vi "VIH HelpGen - Write HTML File - Poly VI.vi"(6 "Owning Palette":cluster{"Name":string, "HTML Path":path}, 8 "error in":errorcluster, 9 "HTML Path":path, 10 "VI Path":path, 11 "Project Tree":T1) -> (0 "error out":errorcluster, 3 "dup Project Tree":T1)   [LabVIEW 2014]
doc: "::: VI Helpeks :::\nCopyright (c) 2000-2026 Konstantin Shifershteyn. All rights reserved."
uses:
  _VIH Project Manager.llb/VIH Project Tree Typedef - Tree Refnum.ctl
panel:
  # "VI Helpeks\nCopyright (c) 2012-2026 Konstantin Shifershteyn"
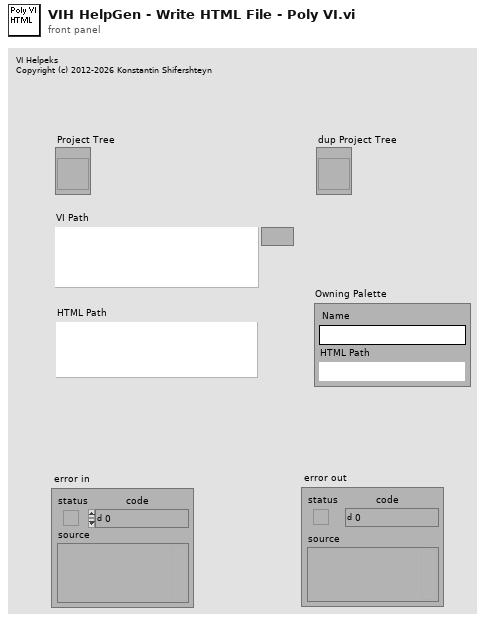
[diagram p1: front panel]
types:
  T1 = typedef "VIH Project Tree Typedef - Tree Refnum.ctl" = refnum<vi>
  T2 = typedef "VIH HelpGen Typedef - Cluster - File Rule.ctl" = cluster{"OutName":string, "BuildHelp":T3, "Source Paths":T4, "Target Paths":T5, "DscrMode":T6, "Description":string, "Control Rules":T7[], "Flags":T9, "Ctl_DscrMode":T6, "Ctl_ClustMembers":T3, "Ctl_EnumValues":T3, "MenuItemIcons":T3, "%Comments":string, "DetailsMode":T6, "DetailsText":string, "ProductInfoMode":T3, "ProductInfoText":string}
  T3 = typedef "VIH HelpGen Typedef - Enum - Default,Enable,Disable.ctl" = enum16{"Default", "Enable", "Disable"}
  T4 = typedef "VIH HelpGen Typedef - Cluster - File Rule - Source Paths.ctl" = cluster{"CSS Files":path[], "JS Files":path[], "Html Template":path}
  T5 = typedef "VIH HelpGen Typedef - Cluster - File Rule - Target Paths.ctl" = cluster{"HTML Dir":path, "Image Dir":path, "CSS Dir":path, "JS Dir":path}
  T6 = typedef "VIH HelpGen Typedef - Enum - Description Mode.ctl" = enum16{"Default", "Description", "Description1", "Description2", "Custom", "None"}
  T7 = typedef "VIH HelpGen Typedef - Cluster - Control Rule.ctl" = cluster{"CtrlID":string, "CustomRule":bool, "DscrMode":T6, "Description":string, "ClusterMembers":T3, "EnumValues":T3, "EnumValDscr":T8[], "CustomName":string}
  T8 = typedef "VIH HelpGen Typedef - Cluster - Enum Value Info.ctl" = cluster{"Value":ext, "String":string, "Description":string}
  T9 = typedef "VIH HelpGen Typedef - Cluster - Group Rule - Flags.ctl" = cluster{"Override CSS Files":bool, "Override JS Files":bool, "Override Ctl Rules":bool}
  T10 = cluster{"ProductInfoMode":T3, "ProductInfoText":string}
  T11 = typedef "VIH HelpGen Typedef - Table Templates Cluster - VI Help.ctl" = cluster{"Ctrl Dscr":string, "Ring Val Dscr":string, "Enum Val Dscr":string, "VI Details":string}
  T12 = cluster{"VI Instance Dscr":string, "Table Templates":T11}
  T13 = cluster{"directory path out":path, "directory path out":path, "name":string}
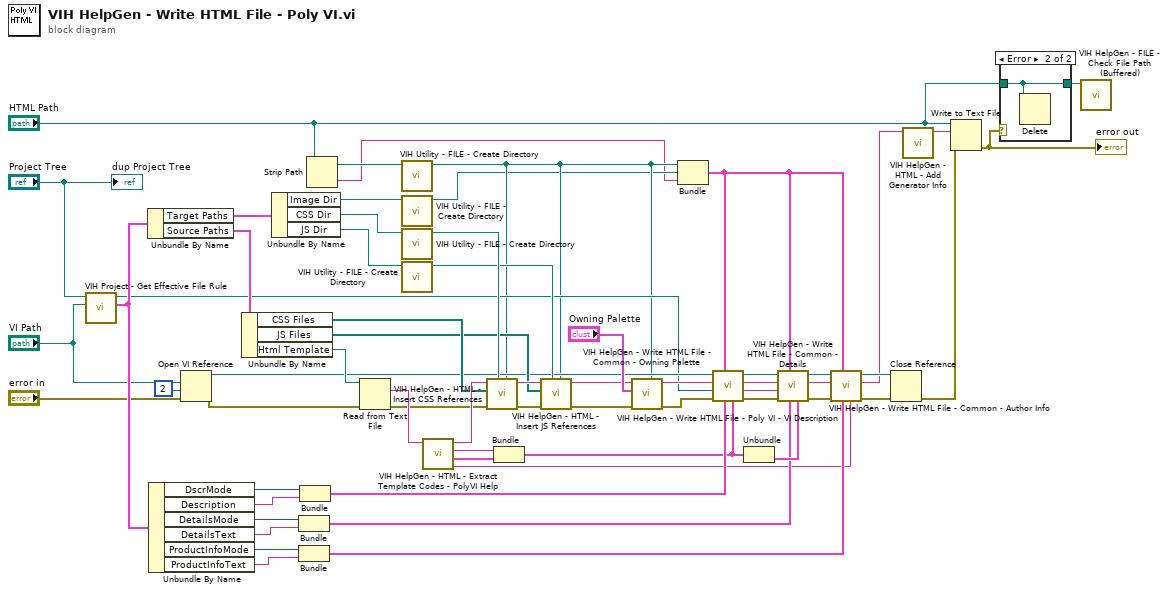
[diagram p0: block diagram]
diagram:
  n1 = call "VIH Project - Get Effective File Rule.vi"("File Path"="VI Path", "Project Tree"="Project Tree") -> ("Effective File Rule"=w48:T2, "dup Project Tree"=w29:T1)  [unwired: 6 in, 2 out]
  n2 = Unbundle By Name(w48) -> ("Target Paths"=w60:T5, "Source Paths"=w59:T4)
  n3 = Unbundle By Name(w48) -> ("DscrMode"=w47:T6, "Description"=w46:string, "DetailsMode"=w22:T6, "DetailsText"=w21:string, "ProductInfoMode"=w8:T3, "ProductInfoText"=w7:string)
  n4 = Open VI Reference(vi path="VI Path", options=2, error in (no error)="error in") -> (vi reference=w35:refnum<vi>, error out=w34:errorcluster)  [unwired: 3 in]
  n5 = Unbundle By Name(w59) -> ("CSS Files"=w58:path[], "JS Files"=w38:path[], "Html Template"=w57:path)
  n6 = Unbundle By Name(w60) -> ("Image Dir"=w49:path, "CSS Dir"=w51:path, "JS Dir"=w44:path)
  n7 = Bundle("DetailsMode"=w22, "DetailsText"=w21) -> (w20:cluster{"DetailsMode":T6, "DetailsText":string})  [unwired: 1 in]
  n8 = Bundle("ProductInfoMode"=w8, "ProductInfoText"=w7) -> (w6:T10)  [unwired: 1 in]
  n9 = Bundle("DscrMode"=w47, "Description"=w46) -> (w45:cluster{"DscrMode":T6, "Description":string})  [unwired: 1 in]
  n10 = Strip Path(path="HTML Path") -> (stripped path=w52:path, name=w1:string)
  n11 = Read from Text File(file (use dialog)=w57, error in=w34) -> (text=w62:string, error out=w56:errorcluster)  [unwired: 2 in, 2 out]
  n12 = call "VIH Utility - FILE - Create Directory.vi"("directory path"=w52) -> ("directory path out"=w4:path)  [unwired: 6 in, 2 out]
  n13 = call "VIH Utility - FILE - Create Directory.vi"("directory path"=w49) -> ("directory path out"=w3:path)  [unwired: 6 in, 2 out]
  n14 = call "VIH Utility - FILE - Create Directory.vi"("directory path"=w51) -> ("directory path out"=w50:path)  [unwired: 6 in, 2 out]
  n15 = call "VIH Utility - FILE - Create Directory.vi"("directory path"=w44) -> ("directory path out"=w39:path)  [unwired: 6 in, 2 out]
  n16 = call "VIH HelpGen - HTML - Extract Template Codes - PolyVI Help.vi"("HTML in"=w62) -> ("ProductInfo Template"=w5:string, "Table Templates"=w30:T11, "VI Instance Dscr"=w31:string, "HTML out"=w61:string)  [unwired: 7 in]
  n17 = call "VIH HelpGen - HTML - Insert CSS References.vi"("HTML Folder"=w4, "CSS Folder"=w50, "error in"=w56, "CSS files"=w58, "HTML in"=w61) -> ("error out"=w42:errorcluster, "HTML out"=w43:string)  [unwired: 5 in]
  n18 = Bundle("VI Instance Dscr"=w31, "Table Templates"=w30) -> (w24:T12)  [unwired: 1 in]
  n19 = call "VIH HelpGen - HTML - Insert JS References.vi"("HTML Folder"=w4, "JSS Folder"=w39, "error in"=w42, "JS files"=w38, "HTML in"=w43) -> ("error out"=w41:errorcluster, "HTML out"=w40:string)  [unwired: 5 in]
  n20 = call "VIH HelpGen - Write HTML File - Common - Owning Palette.vi"("HTML Folder"=w4, "error in"=w41, "Owning Palette"="Owning Palette", "HTML in"=w40) -> ("error out"=w54:errorcluster, "HTML out"=w55:string)  [unwired: 6 in]
  n21 = Bundle("directory path out"=w4, "directory path out"=w3, "name"=w1) -> (w2:T13)  [unwired: 1 in]
  n22 = call "VIH HelpGen - Write HTML File - Poly VI - VI Description.vi"("Templates"=w24, "Description Params"=w45, "Save params"=w2, "error in"=w54, "Project Tree"=w29, "HTML in"=w55, "VI Reference"=w35) -> ("error out"=w25:errorcluster, "VI Name"=w26:string, "HTML out"=w27:string, "dup VI Reference"=w28:refnum<vi>)  [unwired: 1 in]
  n23 = Unbundle(w24) -> ("Table Templates"=w23:T11)  [unwired: 1 out]
  n24 = call "VIH HelpGen - Write HTML File - Common - Details.vi"("Templates"=w23, "Details Params"=w20, "Save params"=w2, "error in"=w25, "Original VI Name"=w26, "HTML in"=w27, "VI Reference"=w28) -> ("error out"=w12:errorcluster, "HTML out"=w13:string, "dup VI Reference"=w14:refnum<vi>)  [unwired: 2 in]
  n25 = call "VIH HelpGen - Write HTML File - Common - Author Info.vi"("Product Info Template"=w5, "Product Info"=w6, "Save params"=w2, "error in"=w12, "HTML in"=w13, "VI Reference"=w14) -> ("error out"=w9:errorcluster, "HTML out"=w10:string, "dup VI Reference"=w11:refnum<vi>)  [unwired: 3 in]
  n26 = Close Reference(reference=w11, error in (no error)=w9) -> (error out=w33:errorcluster)
  n27 = call "VIH HelpGen - HTML - Add Generator Info.vi"("HTML in"=w10) -> ("HTML out"=w16:string)  [unwired: 10 in]
  n28 = Write to Text File(file (use dialog)="HTML Path", text=w16, error in=w33) -> (error out=w18:errorcluster)  [unwired: 1 in, 2 out]
  "error out" <- w18
  n29 = case shown="Error" w18 {
    tunnel: "HTML Path" -> [w63 w64]
    tunnel: [w63 w64] -> w17
    frame No Error {
    }
    frame Error {
      n30 = Delete(path (use dialog)=w64) -> ()  [unwired: 4 in, 3 out]
    }
  }
  n31 = call "VIH HelpGen - FILE - Check File Path (Buffered).vi"("File Path"=w17) -> ()  [unwired: 9 in, 2 out]
  "dup Project Tree" <- "Project Tree"
